vi "DSS-Tests-golden_check.vi"(6 "folder":string="golden", 7 "abs tol":dbl, 8 "error in":errorcluster, 9 "rel tol":dbl=1e-12, 10 "actual":dbl[](array[numeric]), 11 "golden name":string) -> (0 "error out":errorcluster, 2 "message":string, 3 "pass":bool)   [LabVIEW 2020, in "DSS-Tests.lvlib"]
doc: "Checks an actual 1D DBL array against the golden file <tests folder>\\<folder>\\<golden name>.txt; with the marker file goldenæPTURE present (and folder golden) it writes the file instead and passes, so goldens are captured from the current code."
uses:
  DSS-Tests.lvlib
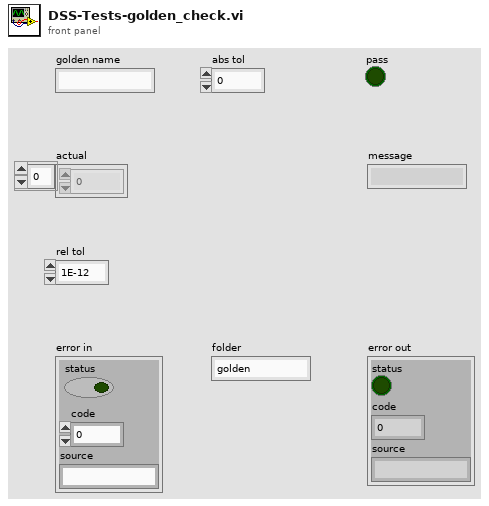
[diagram p1: front panel]
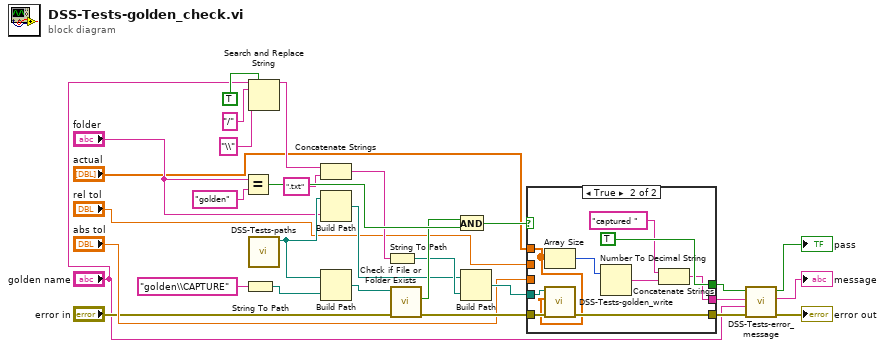
[diagram p0: block diagram]
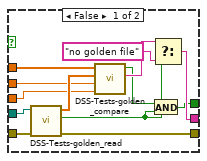
[diagram p2: hidden frame]
diagram:
  n1 = Equal?(x="folder", y="golden" ("golden")) -> (x = y?=w23:bool)
  n2 = String To Path(string="golden\\CAPTURE" ("marker")) -> (path=w18:path)
  n3 = Search and Replace String(replace all?=TRUE ("replace all"), input string="golden name", search string="/" ("slash"), replace string="\\" ("backslash")) -> (result string=w12:string)  [unwired: 4 in, 3 out]
  n4 = call "DSS-Tests-paths.vi"() -> ("tests folder"=w7:path)  [unwired: 10 in, 1 out]
  n5 = Concatenate Strings(w12, ".txt" ("txt")) -> (w14:string)
  n6 = Build Path(base path=w7, name or relative path="folder") -> (appended path=w8:path)
  n7 = Build Path(base path=w7, name or relative path=w18) -> (appended path=w19:path)
  n8 = String To Path(string=w14) -> (path=w15:path)
  n9 = call <vilib>:"Check if File or Folder Exists.vi"("error in (no error)"="error in", "path"=w19) -> ("error out"=w20:errorcluster, "file or folder exists?"=w21:bool)  [unwired: 7 in, 1 out]
  n10 = And(x=w21, y=w23) -> (x .and. y?=w24:bool)
  n11 = Build Path(base path=w8, name or relative path=w15) -> (appended path=w16:path)
  n12 = case shown="True" w24 {
    tunnel: "actual" -> [w32 w45]
    tunnel: "rel tol" -> [w34 _]
    tunnel: "abs tol" -> [w35 _]
    tunnel: [w41 TRUE ("pass true")] -> w25
    tunnel: w20 -> [w33 w46]
    tunnel: w16 -> [w31 w44]
    tunnel: [w43 w51] -> w26
    tunnel: [w38 w47] -> w27
    frame False {
      n13 = call "DSS-Tests-golden_read.vi"("error in"=w33, "file path"=w31) -> ("error out"=w38:errorcluster, "found"=w37:bool, "values"=w36:dbl[])  [unwired: 7 in]
      n14 = call "DSS-Tests-golden_compare.vi"("abs tol"=w35, "rel tol"=w34, "golden"=w36, "actual"=w32) -> ("message"=w40:string, "pass"=w39:bool)  [unwired: 5 in, 1 out]
      n15 = And(x=w39, y=w37) -> (x .and. y?=w41:bool)
      n16 = Select(t=w40, s=w37, f="no golden file" ("t no golden")) -> (s? t:f=w43:string)
    }
    frame True {
      n17 = Array Size(array=w45) -> (size(s)=w48:i32)
      n18 = call "DSS-Tests-golden_write.vi"("error in"=w46, "values"=w45, "file path"=w44) -> ("error out"=w47:errorcluster)  [unwired: 8 in]
      n19 = Number To Decimal String(number=w48) -> (decimal integer string=w49:string)  [unwired: 1 in]
      n20 = Concatenate Strings("captured " ("t captured"), w49) -> (w51:string)
    }
  }
  n21 = call "DSS-Tests-error_message.vi"("error in"=w27, "prefix"="golden name", "message in"=w26, "pass in"=w25) -> ("error out"=→"error out":errorcluster, "message"=→"message":string, "pass"=→"pass":bool)  [unwired: 5 in]
